vi "Native_GetControlTerminal.vi"() -> ()   [LabVIEW 2024]
panel:
  out "error out":errorcluster caption="错误输出"
  out "terminal_id":u32
  in  "terminal_id type":u32
  in  "control_id":u32
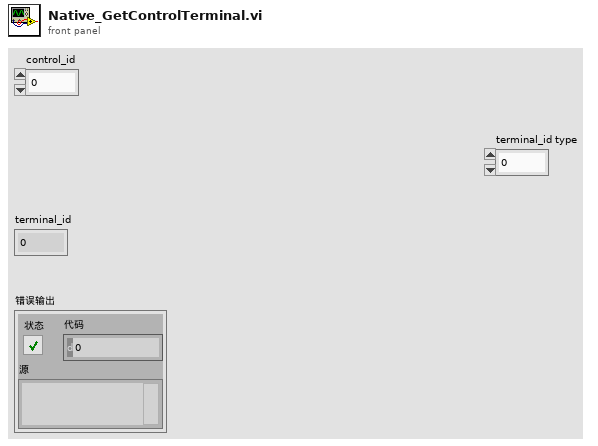
[diagram p1: front panel]
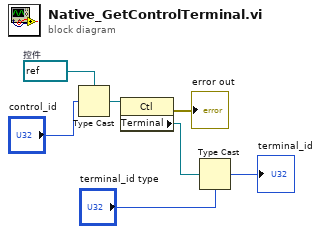
[diagram p0: block diagram]
diagram:
  w6 = refnum<vi> refnum  # 控件
  n1 = Type Cast ("强制类型转换")(type=w6, x="control_id") -> (*(type *) &x=w5:refnum<vi>)
  n2 = property on="属性节点" class="Ctl"(reference=w5) -> (error out=→"error out":errorcluster, "Terminal"=w4:refnum<vi>)  [unwired: 1 in, 1 out]
  n3 = Type Cast ("强制类型转换")(type="terminal_id type", x=w4) -> (*(type *) &x=→"terminal_id":u32)
